vi "OPC Read All.vi"(0 "Init":bool, 3 "Ctl":refnum<vi>[](array[refnum]), 5 "错误输入（无错误）":errorcluster, 8 "update":bool, 9 "queue array in":refnum<queue>[](array[refnum])) -> (10 "write":u8[](array[numeric]), 11 "Error":cluster{i32, i32, string[]}, 14 "Comm ok?":bool, 16 "State":T1 {"托盘类型" items=["NONE", "CMA", "XP", "IEM", "BEV", "GAC", "MEP2"]}, 17 "Read":u8[](array[numeric]), 19 "error out":errorcluster)   [LabVIEW 2012]
uses:
  Globals/Global.vi
  Queue VIs/Type define/element data type.ctl
  Config/Ctl/OPC Read 1.ctl
panel:
  # "线体"
  # "Buffer区"
  # "顶升平移机构"
  # "电控箱"
  # "Buffer区"
  # "顶升平移机构"
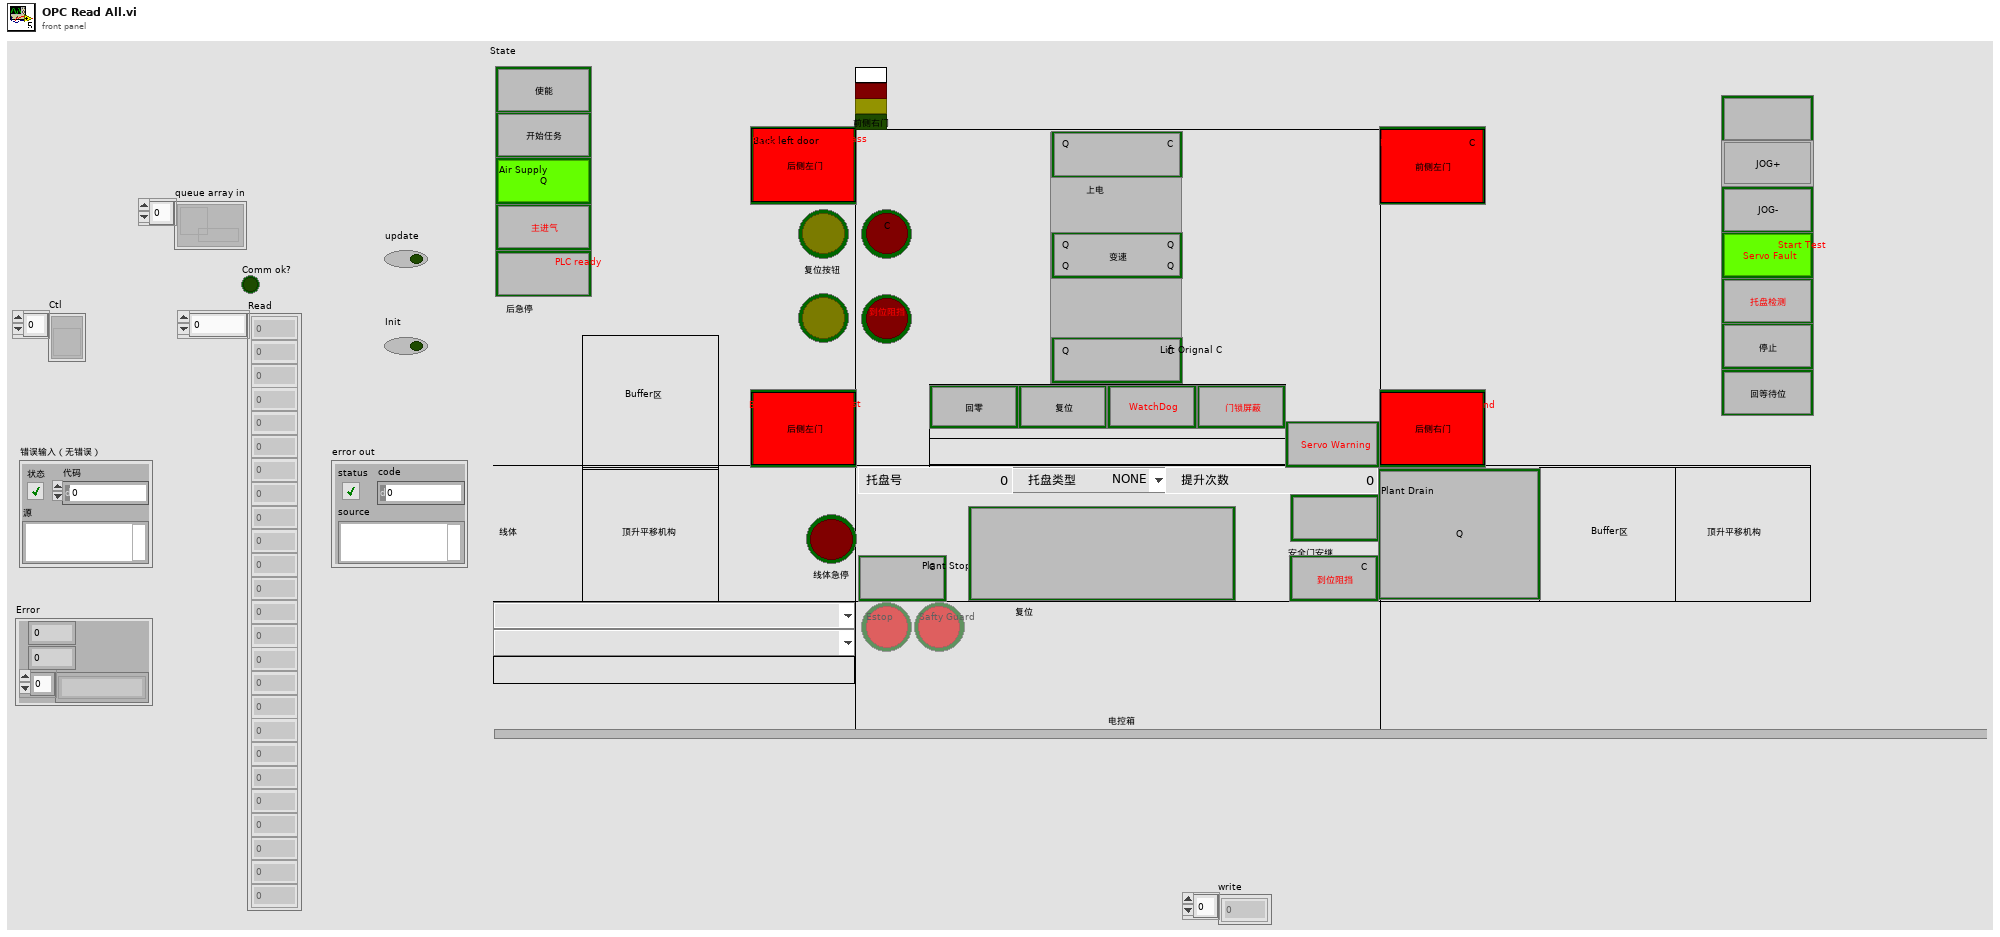
[diagram p1: front panel]
types:
  T1 = typedef "OPC Read 1.ctl" = cluster{"Cycle Time":u32, "Barcode":string, "托盘类型":i64, "提升次数":i64, "托盘号":i16, "Back left door":bool, "Front left door":bool, "Back Right door":bool, "Front Right door":bool, "LED G":bool, "LED Y":bool, "LED R":bool, "LED W":bool, "Reset BT":bool, "Reset LED":bool, "Plant Stop":bool, "Plant Stop C":bool, "Safty Guard":bool, "Estop":bool, "Front Estop":bool, "Back Estop":bool, "Lift Work Input":bool, "Plant Check":bool, "Lift Orignal Input":bool, "WDT":bool, "Door F":bool, "PLC Ready":bool, "PLC Alarm":bool, "PC Alarm":bool, "PC Warning":bool, "PLC Stop":bool, "Bypass":bool, "PLC Start":bool, "Auto Mode":bool, "Start Test":bool, "In Test":bool, "In End":bool, "In Pass":bool, "In Fail":bool, "Door F C":bool, "AutoStep":i64, "InitialStep":i64, "StepMsg":string, "Back left door Q":bool, "Front left door Q":bool, "Back Right door Q":bool, "Front Right door Q":bool, "Product Check":bool, "Auto Mode C":bool, "Left Front Door C":bool, "Right Front Door C":bool, "Left Back Door C":bool, "Right back Door C":bool, "Lift Work C":bool, "Lift Orignal C":bool, "Air Supply":bool, "Plant Drain":bool, "Comm Timeout":bool, "Line Estop":bool, "Lift Speed":bool, "Lift Work Q":bool, "Lift Orignal Q":bool, "Plant Stop 2":bool, "Plant Stop C 2":bool, "UP F Q":bool, "UP S Q":bool, "DOWN F Q":bool, "DOWN S Q":bool}
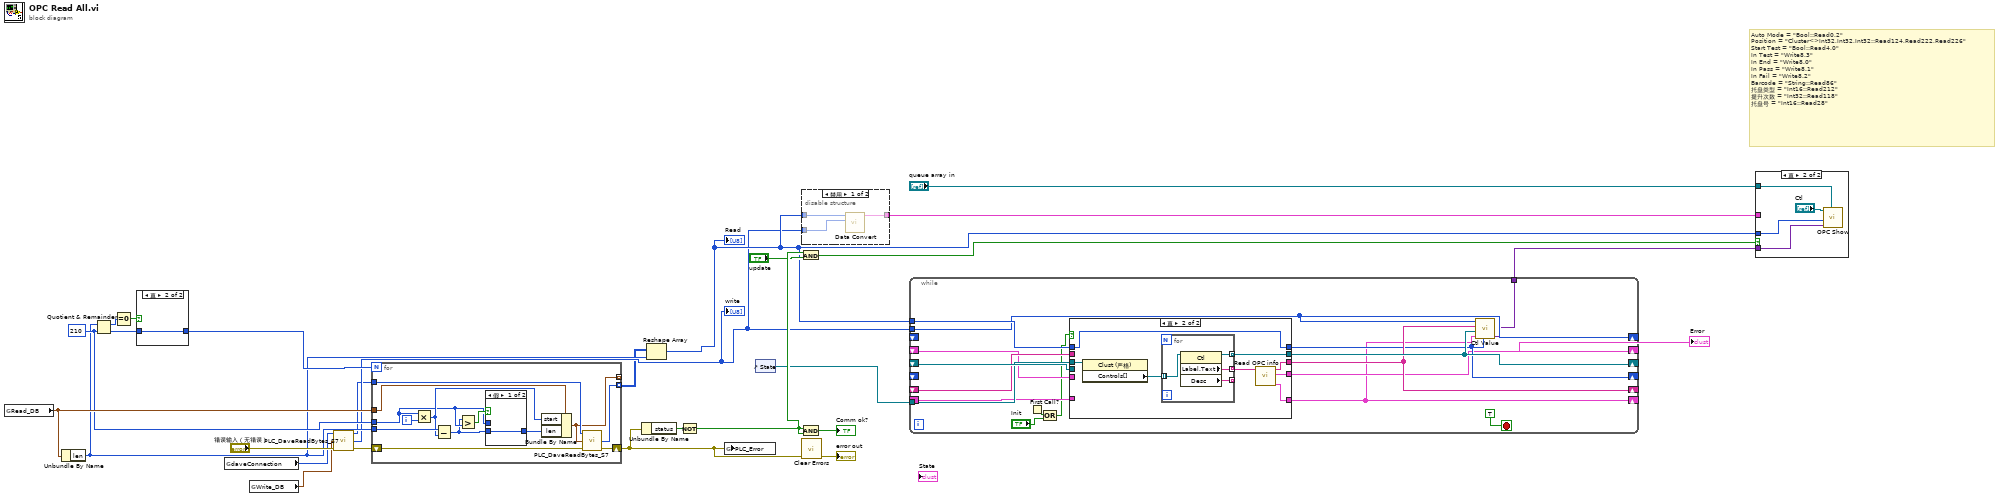
[diagram p0: block diagram]
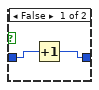
[diagram p3: hidden frame]
diagram:
  w9 = 210 ("y")
  # "Auto Mode = \"Bool::Read0.2\"\nPosition = \"Cluster<>Int32,Int32,Int32::Read124,Read222,Read226\"\nStart Test = \"Bool::Read4.0\"\nIn Test = \"Write8.3\"\nIn End = \"Write8.0\"\nIn Pass = \"Write8.1\"\nIn Fail = \"Write8.2\"\nBarcode = \"String::Read86\"\n托盘类型 = \"Int16::Read212\"\n提升次数 = \"Int32::Read118\"\n托盘号 = \"Int16::Read28\""
  n1 = global read "Global.vi" "Read_DB"() -> (w14:cluster{"DB":i32, "start":i32, "len":i32})
  n2 = Unbundle By Name(w14) -> ("len"=w8:i32)
  n3 = Quotient & Remainder(x=w8, y=w9) -> (x-y*floor(x/y)=w13:i32, floor(x/y)=w11:i32)
  n4 = Equal To 0?(x=w13) -> (x = 0?=w12:bool)
  n5 = case shown="真" w12 {
    tunnel: w11 -> [w29 w30]
    tunnel: [w28 w30] -> w10
    frame False {
      n6 = Increment(x=w29) -> (x+1=w28:i32)
    }
    frame True {
    }
  }
  n7 = global read "Global.vi" "daveConnection"() -> (w21:i64)
  n8 = global read "Global.vi" "Write_DB"() -> (w18:cluster{"DB":i32, "start":i32, "len":i32})
  n9 = call "PLC_DaveReadBytes_S7.vi"("daveConnection in"=w21, "地址"=w18, "error in (no error)"="错误输入（无错误）") -> ("daveConnection out"=w5:i64, "read Buffer"=w6:u8[], "error out"=w4:errorcluster)  [unwired: 9 in, 1 out]
  "write" <- w6
  n10 = for {
    N: w10 -> [_]
    tunnel: w5 -> [w43]
    tunnel: [w41] -> w3 mode=indexing
    tunnel: w14 -> [w38]
    shift-right: [w40] -> w19
    shift-left: w4 -> [w42]
    tunnel: w9 -> [w32]
    tunnel: [w37] -> _ mode=indexing
    tunnel: w8 -> [w36]
    i -> [w39]
    n11 = Multiply(x=w32, y=w39) -> (x*y=w35:i32)
    n12 = Subtract(x=w36, y=w35) -> (x-y=w31:i32)
    n13 = Greater?(x=w31, y=w32) -> (0:w34:bool)
    n14 = case shown="假" w34 {
      tunnel: [w44 w45] -> w33
      tunnel: w32 -> [_ w45]
      tunnel: w31 -> [w44 _]
      frame False {
      }
      frame True {
      }
    }
    n15 = Bundle By Name(cluster=w38, "start"=w35, "len"=w33) -> (w37:cluster{"DB":i32, "start":i32, "len":i32})
    n16 = call "PLC_DaveReadBytes_S7.vi"("daveConnection in"=w43, "地址"=w37, "error in (no error)"=w42) -> ("read Buffer"=w41:u8[], "error out"=w40:errorcluster)  [unwired: 9 in, 2 out]
  }
  n17 = Unbundle By Name(w19) -> ("status"=w2:bool)
  n18 = Reshape Array(w3, w8) -> (w16:u8[])
  "Read" <- w16
  n19 = Not(x=w2) -> (.not. x?=w26:bool)
  n20 = global write "Global.vi" "PLC_Error"(w19) -> ()
  n21 = control-ref of="State"() -> (w15:refnum<vi>)
  n22 = And(x=w26, y="update") -> (x .and. y?=w22:bool)
  n23 = And(x=w26, y=w26) -> (x .and. y?=→"Comm ok?":bool)
  n24 = disable-structure shown="禁用" {
    disable-tunnel: w6 -> [w48 _]
    disable-tunnel: [w47 _] -> w24
    disable-tunnel: w16 -> [w46 _]
    frame Disabled {
      n25 = call "Data Convert.vi"("write data"=w48, "read data"=w46) -> ("State"=w47:T1)  [unwired: 9 in]
    }
    frame Enabled {
    }
  }
  n26 = call <vilib>:"Clear Errors.vi"("error in (no error)"=w19) -> ("error out"=→"error out":errorcluster)  [unwired: 5 in, 1 out]
  n27 = while {
    shift-right: [w62] -> _
    shift-left: _ -> [w65]
    shift-right: [w61] -> _
    shift-left: _ -> [w63]
    tunnel: w16 -> [w64]
    shift-right: [w59] -> _
    shift-left: _ -> [_]
    shift-right: [w58] -> _
    shift-left: _ -> [_]
    tunnel: w6 -> [w58]
    tunnel: w15 -> [w57]
    shift-right: [w56] -> w7
    shift-left: _ -> [w55]
    shift-right: [w53] -> _
    shift-left: _ -> [w54]
    tunnel: [w52] -> w1
    stop <- TRUE stop-if-true
    n28 = First Call?() -> (First Call?: T/F=w50:bool)
    n29 = Or(x=w50, y="Init") -> (x .or. y?=w49:bool)
    n30 = case shown="真" w49 {
      tunnel: [w70 w76] -> w62
      tunnel: w65 -> [w70 _]
      tunnel: [w69 w78] -> w59
      tunnel: w64 -> [w69 w78]
      tunnel: [w68 w74] -> w61
      tunnel: w63 -> [w68 _]
      tunnel: w57 -> [_ w73]
      tunnel: [w67 w72] -> w56
      tunnel: w55 -> [w67 _]
      tunnel: [w66 w71] -> w53
      tunnel: w54 -> [w66 _]
      frame False {
      }
      frame True {
        n31 = property class="Clust (严格)"(reference=w73) -> ("Controls[]"=w77:refnum<vi>[])  [unwired: 1 in, 2 out]
        n32 = for {
          tunnel: w77 -> [w82] mode=indexing
          tunnel: [w81] -> w76 mode=indexing
          tunnel: [w80] -> _ mode=indexing
          tunnel: [w79] -> w75 mode=indexing
          n33 = property class="Ctl"(reference=w82) -> (reference out=w81:refnum<vi>, "Label.Text"=w79:string, "Desc"=w80:string)  [unwired: 1 in, 1 out]
        }
        n34 = call "Read OPC info.vi"("Read ctl"=w75) -> ("Value Event"=w71:cluster{"String":string, "value":string}[], "Error"=w72:cluster{i32, i32, string[]}, "Read"=w74:string[])  [unwired: 7 in, 1 out]
      }
    }
    n35 = call "Ctl Value.vi"("read Buffer 2"=w59, "Value Event"=w53, "数组"=w62, "Read"=w61, "read Buffer"=w58) -> ("Value"=w52:variant[])  [unwired: 6 in]
  }
  "Error" <- w7
  n36 = case shown="真" w22 {
    tunnel: "queue array in" -> [_ w86]
    tunnel: w16 -> [_ w85]
    tunnel: w24 -> [_ _]
    tunnel: w1 -> [_ w83]
    frame False {
    }
    frame True {
      n37 = call "OPC Show.vi"("queue array in"=w86, "Value"=w83, "Read"=w85, "Ctl In"="Ctl") -> ()  [unwired: 8 in]
    }
  }
